vi "Set Pulse Cycle.vi"(8 "error in (no error)":errorcluster caption="错误输入（无错误）", 9 "nCycle":i32, 10 "nBoard":i32, 11 "nDevId":i32) -> (0 "error out":errorcluster caption="错误输出", 3 "function return":i32)   [LabVIEW 2017, in "smncsftmt.lvlib"]
doc: "__declspec(dllexport) int SetPulseCycle(int nDevId, int nBoard, int nCycle);"
uses:
  smncsftmt.lvlib
  smncsftmt.dll
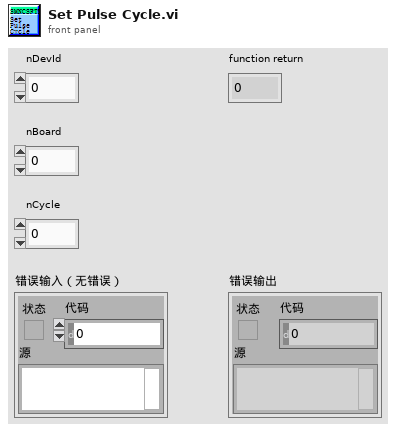
[diagram p1: front panel]
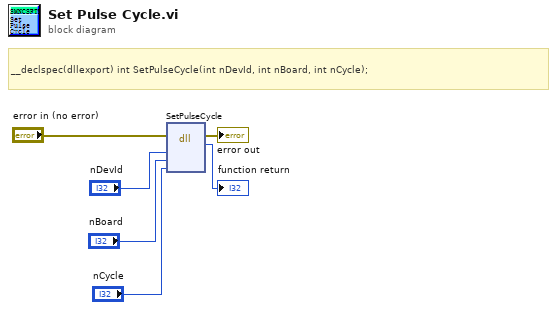
[diagram p0: block diagram]
diagram:
  # "__declspec(dllexport) int SetPulseCycle(int nDevId, int nBoard, int nCycle);"
  n1 = dll-call lib="PTH2oabs CUsersaDesktop\nLABVIEW范例National InstrumentsLabVIEW 2017user.lib\tsmncsftmtsmncsftmt.*" fn="SetPulseCycle"(error in="error in (no error)", "nDevId"="nDevId", "nBoard"="nBoard", "nCycle"="nCycle") -> (error out=→"error out":errorcluster, →"function return":i32)  [unwired: 5 in, 1 out]
